vi "Compute.vi"(7 "SHA-1":refnum<class "SHA-1.lvclass">, 10 "data":u8[](array[numeric]) format="%02x") -> (2 "hash":u8[](array[numeric]) format="%02x")   [LabVIEW 2013, in "SHA-1.lvlib" / "SHA-1.lvclass"]
doc: "This VI contains the core of the MD5 algorithm."
uses:
  SHA-1.lvclass
  Data-vector.ctl
  pad.vi
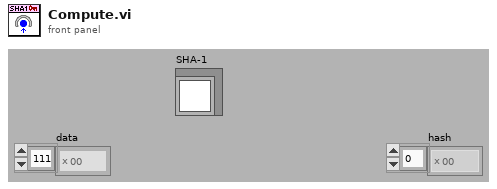
[diagram p1: front panel]
types:
  T1 = typedef "SHA-1.lvlib/SHA-1.lvclass/Data-vector.ctl" = cluster{"Data[ ]":u8[], "end":bool}
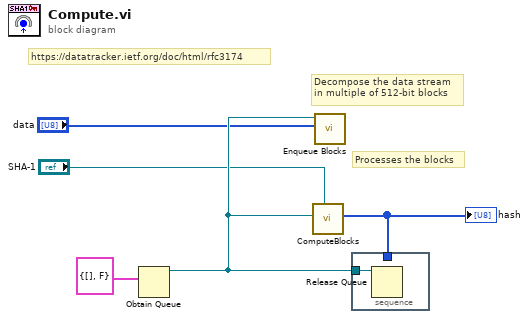
[diagram p0: block diagram]
diagram:
  # "Processes the blocks"
  # "Decompose the data stream\nin multiple of 512-bit blocks"
  # "https://datatracker.ietf.org/doc/html/rfc3174"
  n1 = Obtain Queue(element data type=T1 {"Data[ ]"=[], "end"=FALSE} ("cluster")) -> (queue out=w4:refnum<queue>)  [unwired: 4 in, 2 out]
  n2 = call-dynamic "ComputeBlocks.vi"("SHA-1"="SHA-1", "blocks queue"=w4) -> ("hash"=w2:u8[])  [unwired: 9 in]
  "hash" <- w2
  n3 = call "Enqueue Blocks.vi"("data"="data", "Blocks queue"=w4) -> ()  [unwired: 10 in]
  n4 = stacked-sequence {
    tunnel: w4 -> [w6]
    tunnel: w2 -> [_]
    frame #0 {
      n5 = Release Queue(queue=w6) -> ()  [unwired: 2 in, 3 out]
    }
  }
